vi "PhotonVision_Globals.vi"() -> ()   [LabVIEW 2019, in "PhotonVisionLib.lvlib"]
uses:
  PhotonVisionLib.lvlib
  <vilib>/Rock Robotics/WPI/ThirdParty/JAS_Junk/TrajLib/TypeDef/ROTATION2D.ctl
  <vilib>/Rock Robotics/WPI/ThirdParty/JAS_Junk/TrajLib/Trajectory_Library.lvlib
  <vilib>/Rock Robotics/WPI/ThirdParty/JAS_Junk/TrajLib/TypeDef/TIME_INTERPOLATABLE_ROTATION2D.ctl
panel:
  out "PoseEstimatorHeadingBuffer":T1 {"RotationValues"."SIN" format="%13.4f"; "RotationValues"."COS" format="%13.4f"; "RotationValues"."VALUE" format="%13.4f"}
  out "PV_TimeSyncClientLastSentSrcPort":u16
  out "PV_TimeSyncClientLastRcvSrcPort":u16
  out "PV_TimeSyncClientLastRcvIP":u32
  out "PV_TimeSyncServLastSrcPort":u32
  out "PV_TimeSyncClientReadLoopCnt":i32
  out "PV_TimeSyncServRcvIP":u32
  out "PV_TimeSyncClientLastRcvId":i8
  out "PV_TimeSyncClientLastRcvVer":i8
  out "PV_TimeSyncClientReadErr":bool
  out "PV_TimeSyncClientWriteErr":bool
  out "PV_TimeSyncServReadErr":bool
  out "PV_TimeSyncServWriteErr":bool
  out "PV_TimeSyncClientTimeOffset":i64
  out "PV_TimeSyncClientLastRcvTime":i64
  out "PV_TimeSyncClientLoopCnt":i32
  out "PV_TimeSyncClientLastSentTime":i64
  out "PV_TimeSyncClientStop":bool
  out "PV_TimeSyncServLoopCount":i32
  out "PV_TimeSyncServStop":bool
  out "PV_TimeSyncServLastSentTime":i64
  out "PV_TimeSyncServLastRcvTim":i64
  out "PV_TimeSyncServLastRcvId":i8
  out "PV_TimeSyncServLastRcvVer":i8
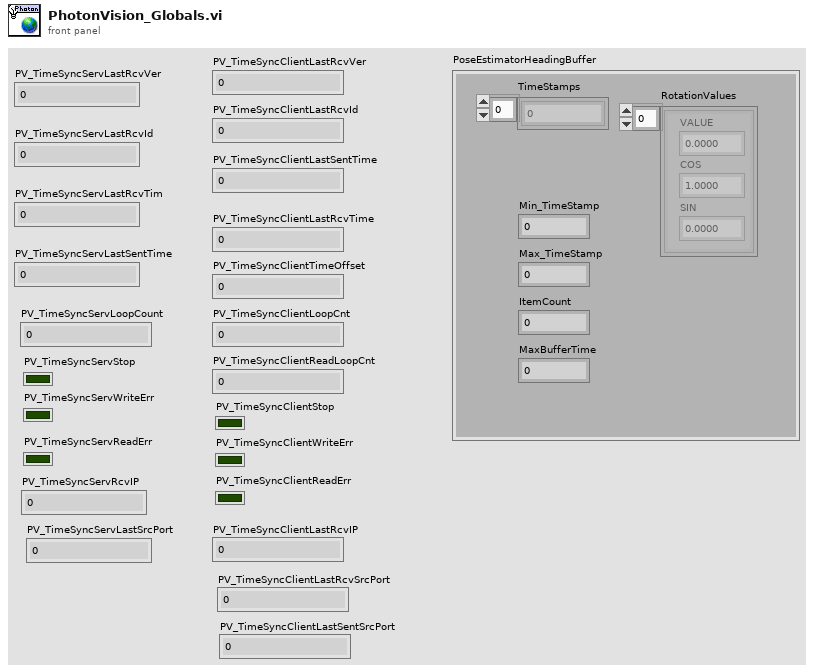
[diagram p1: front panel]
types:
  T1 = typedef "Trajectory_Library.lvlib/TIME_INTERPOLATABLE_ROTATION2D.ctl" = cluster{"TimeStamps":dbl[], "RotationValues":T2[], "Min_TimeStamp":dbl, "Max_TimeStamp":dbl, "ItemCount":i32, "MaxBufferTime":dbl}
  T2 = typedef "Trajectory_Library.lvlib/ROTATION2D.ctl" = cluster{"VALUE":dbl, "COS":dbl, "SIN":dbl}
diagram:
